vi "Set Tree Symbols All.vi"(8 "error in (no error)":errorcluster, 10 "symbol":i32, 11 "Tree Refnum":refnum<vi>) -> (0 "error out":errorcluster, 2 "Seted Tags":T1(array[cluster]), 3 "Tree Refnum":refnum<vi>)   [LabVIEW 2023, in "DSLV_Tree.lvlib"]
uses:
  DSLV_Tree.lvlib
panel:
  # "tips:\nsymbol num:symbol\n37:checkbox unselected\n38:checkbox selected"
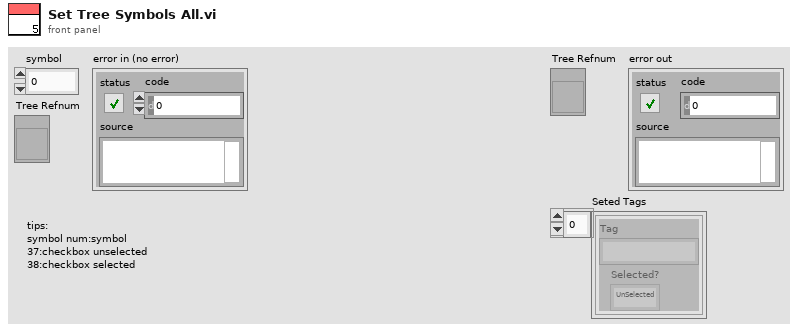
[diagram p1: front panel]
types:
  T1 = cluster{"Tag":string, "Selected?":enum16{"UnSelected", "Selected", "PartSelected"}}[]
  T2 = cluster{"Tag":string, "Selected?":enum16{"UnSelected", "Selected", "PartSelected"}}
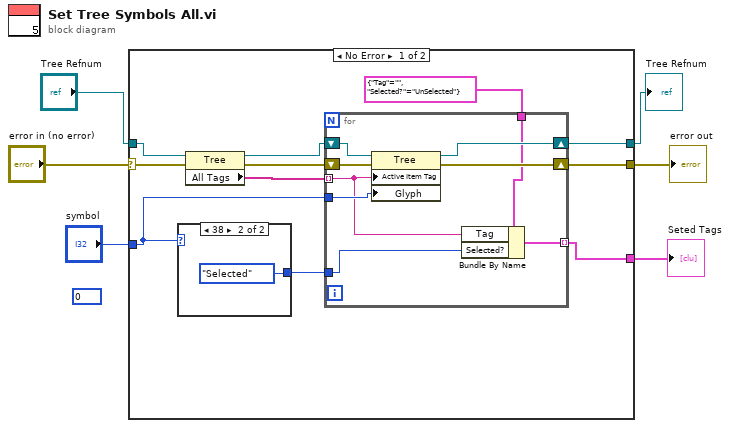
[diagram p0: block diagram]
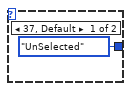
[diagram p2: hidden frame]
diagram:
  (unwired) 0
  n1 = case shown="No Error" "error in (no error)" {
    selector: "error in (no error)" -> [w13 w29]
    tunnel: "symbol" -> [w8 _]
    tunnel: [w15 w30] -> w5
    tunnel: "Tree Refnum" -> [w14 w30]
    tunnel: [w12 w29] -> w3
    tunnel: [w9 _] -> w1
    frame No Error {
      n2 = case shown="38" w8 {
        tunnel: [enum16{"UnSelected", "Selected", "PartSelected"}."UnSelected" ("Selected?") enum16{"UnSelected", "Selected", "PartSelected"}."Selected" ("Selected?")] -> w7
        frame 37, Default {
        }
        frame 38 {
        }
      }
      n3 = property class="Tree"(reference=w14, error in=w13) -> (reference out=w16:refnum<vi>, error out=w17:errorcluster, "All Tags"=w11:string[])
      n4 = for {
        tunnel: w11 -> [w21] mode=indexing
        shift-right: [w25] -> w12
        shift-left: w17 -> [w27]
        shift-right: [w26] -> w15
        shift-left: w16 -> [w28]
        tunnel: w8 -> [w24]
        tunnel: T2 {"Tag"="", "Selected?"=enum."UnSelected"} ("Set") -> [w23]
        tunnel: [w22] -> w9 mode=indexing
        tunnel: w7 -> [w20]
        n5 = property on="Property Node" class="Tree"(reference=w28, error in=w27, "Active Item Tag"=w21, "Glyph"=w24) -> (reference out=w26:refnum<vi>, error out=w25:errorcluster)
        n6 = Bundle By Name(cluster=w23, "Tag"=w21, "Selected?"=w20) -> (w22:T2)
      }
    }
    frame Error {
    }
  }
  "Tree Refnum" <- w5
  "error out" <- w3
  "Seted Tags" <- w1
